vi "TDMSWrite(SubVI)_3ch.vi"(0 "tdms file out 입력":refnum<k34>, 1 "배열":dbl[](array[numeric]), 5 "그룹입력":string="Robot-M1509", 7 "채널입력":string[](array[string]), 11 "에러 입력":errorcluster caption="에러 입력(에러 없음)") -> (4 "참조 번호 출력":refnum<k34>, 15 "에러 출력":errorcluster)   [LabVIEW 2019]
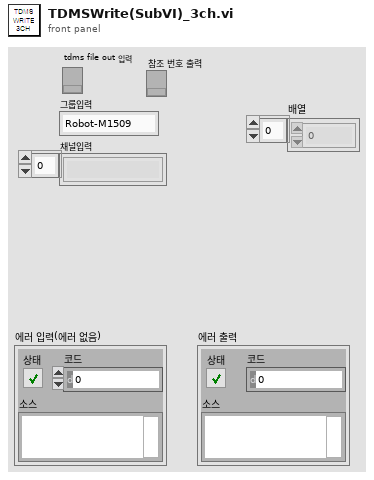
[diagram p1: front panel]
types:
  T1 = cluster{"배열[0]":dbl, "배열[1]":dbl, "배열[2]":dbl, "배열[3]":dbl, "배열[4]":dbl, "배열[5]":dbl, "배열[6]":dbl, "배열[7]":dbl, "배열[8]":dbl}
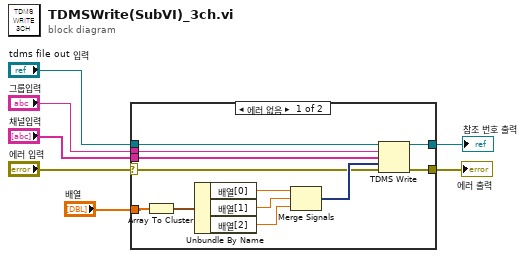
[diagram p0: block diagram]
diagram:
  n1 = case shown="에러 없음" "에러 입력" {
    selector: "에러 입력" -> [w15 w20]
    tunnel: [w18 w21] -> w7
    tunnel: [w17 w20] -> w6
    tunnel: "tdms file out 입력" -> [w16 w21]
    tunnel: "그룹입력" -> [w14 _]
    tunnel: "채널입력" -> [w13 _]
    tunnel: "배열" -> [w12 _]
    frame No Error {
      n2 = Array To Cluster(array=w12) -> (cluster=w11:T1)
      n3 = Unbundle By Name(w11) -> ("배열[0]"=w10:dbl, "배열[1]"=w9:dbl, "배열[2]"=w8:dbl)
      n4 = Merge Signals(w10, w9, w8) -> (w19:dynamicdata)
      n5 = TDMS Write(0:w16, 5:w14, 7:w13, 9:w19, 11:w15) -> (4:w18:refnum<k34>, 15:w17:errorcluster)  [unwired: 1 in, 2 out]
    }
    frame Error {
    }
  }
  "참조 번호 출력" <- w7
  "에러 출력" <- w6
